vi "CaptureWaveDemo.vi"() -> ()   [LabVIEW 2015]
panel:
  out "结果描述":string
  out "csv文件输出路径":string
  out "波形图":sgl[](graph)
  out "数据缓存":u8[](array[numeric])
  in  "读取方式":enum16{"bin", "csv"}(ring)
  out "Dll路径":path
  in  "指令":string(combo)="capture wave:.bin@CH:0@DT:vol;"
  in  "超时(ms)":u32=2000
  in  "设备地址":string="[C:DSO][D:DSO-X][T:USB][PID:0x5537][VID:0x4348][EI:0x82][EO:0x2][CFG:1][I:0]"
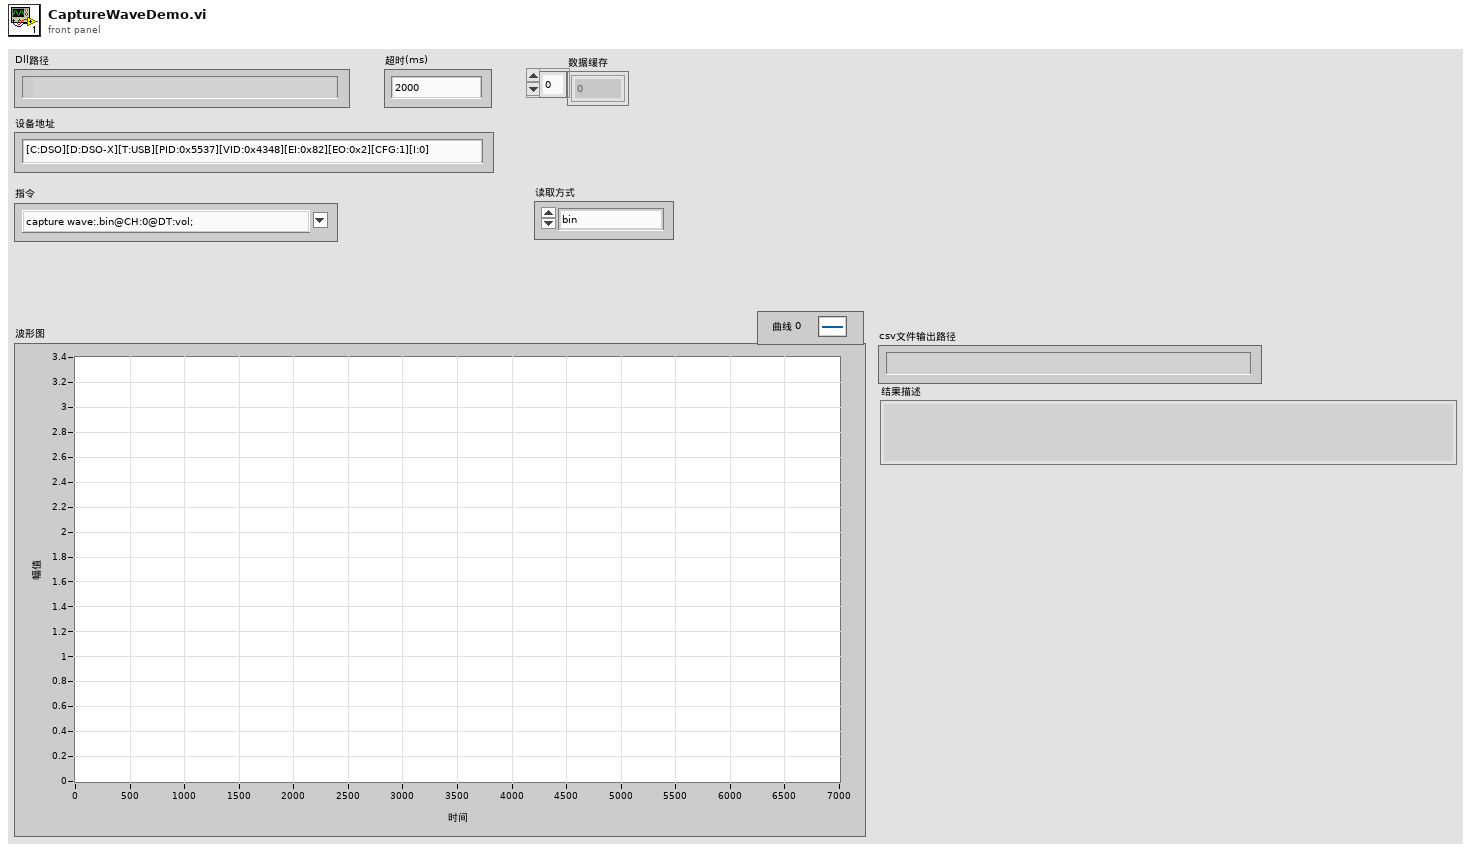
[diagram p1: front panel]
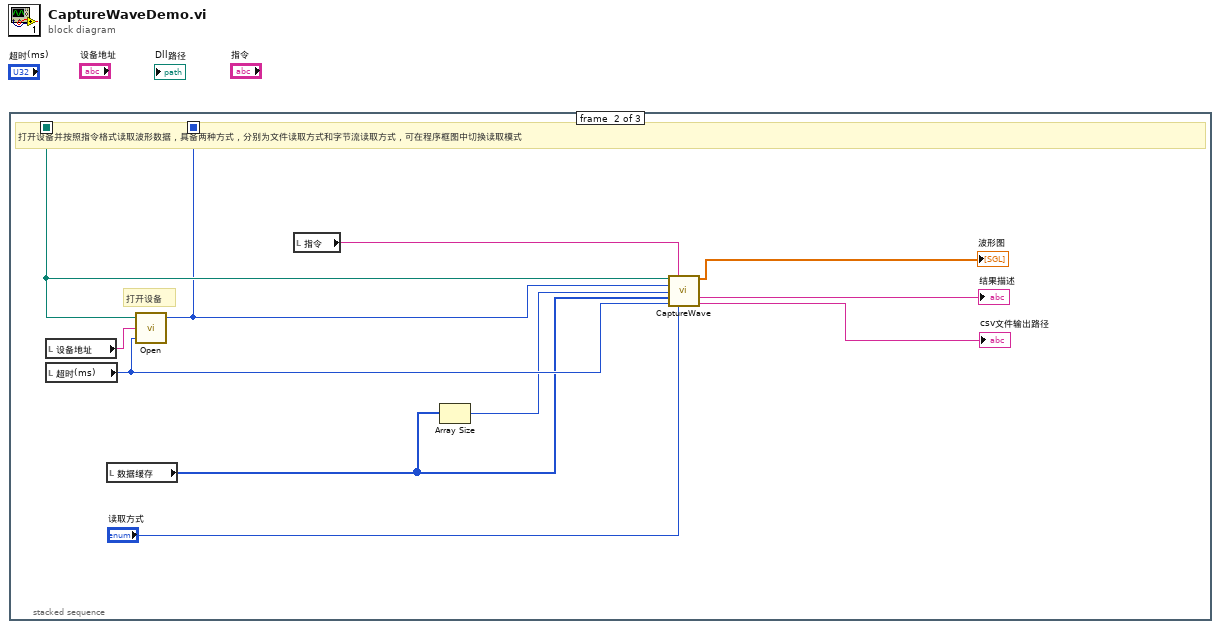
[diagram p0: block diagram]
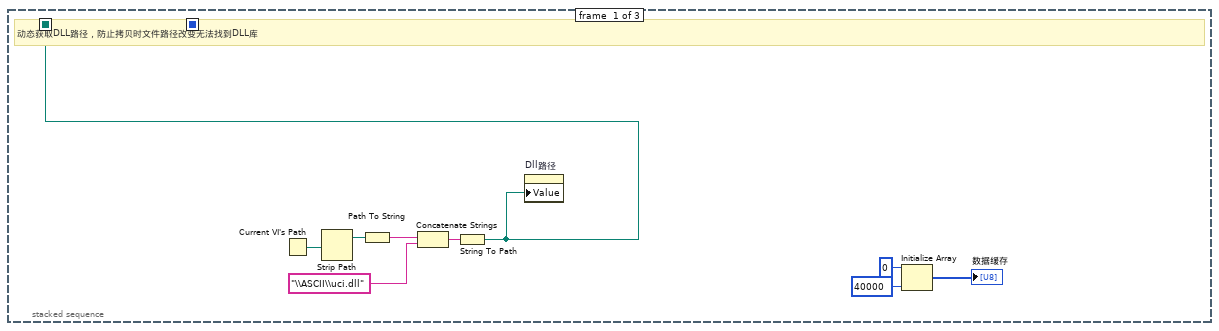
[diagram p2: hidden frame]
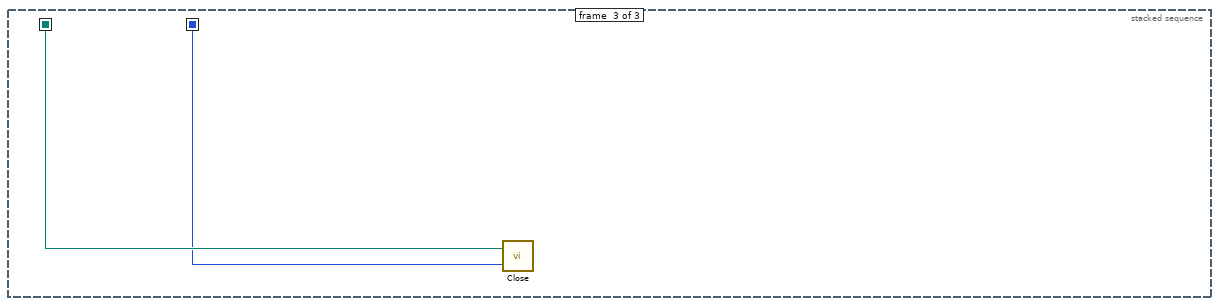
[diagram p3: hidden frame]
diagram:
  n1 = stacked-sequence {
    seq-local: [w4 _ _] -> [_ w17 w22]
    seq-local: [_ w16 _] -> [_ _ w21]
    frame #0 {
      # "动态获取DLL路径，防止拷贝时文件路径改变无法找到DLL库"
      n2 = Current VI's Path() -> (path=w8:path)
      n3 = Strip Path(path=w8) -> (stripped path=w6:path)  [unwired: 1 out]
      n4 = Path To String(path=w6) -> (string=w5:string)
      n5 = Concatenate Strings(w5, "\\ASCII\\uci.dll" ("字符串")) -> (w7:string)
      n6 = String To Path(string=w7) -> (path=w4:path)
      n7 = property on="Dll路径" class="Path"("Value"=w4) -> ()  [unwired: 2 in, 2 out]
      n8 = Initialize Array(u8 0 ("元素"), 40000 ("维数大小")) -> (→"数据缓存":u8[])
    }
    frame #1 {
      # "打开设备"
      # "打开设备并按照指令格式读取波形数据，具备两种方式，分别为文件读取方式和字节流读取方式，可在程序框图中切换读取模式"
      n9 = local read "设备地址"() -> (w20:string)
      n10 = local read "超时(ms)"() -> (w15:u32)
      n11 = local read "数据缓存"() -> (w14:u8[])
      n12 = call "Open.vi"("Timeout"=w15, "Addr"=w20, "UCI_DllPath"=w17) -> ("Session_id"=w16:i32)  [unwired: 2 out]
      n13 = local read "指令"() -> (w18:string)
      n14 = Array Size(array=w14) -> (size(s)=w13:i32)
      n15 = call "CaptureWave.vi"("UCI_DllPath"=w17, "Command"=w18, "Session_id"=w16, "Length"=w13, "InputData"=w14, "Timeout(ms)"=w15, "ReadType"="读取方式") -> ("OutputData"=→"波形图":sgl[], "ResultDescription"=→"结果描述":string, ".csv File Path"=→"csv文件输出路径":string)  [unwired: 6 in]
    }
    frame #2 {
      n16 = call "Close.vi"("Session_id"=w21, "UCI_DllPath"=w22) -> ()  [unwired: 1 out]
    }
  }
